vi "Run TDR.vi"(9 "Apply TDR?":bool, 11 "DPE Project File Path":string) -> (0 "error out":errorcluster, 3 "DPI Instrument Name":refnum<k15>)   [LabVIEW 2025, in "Digital Pattern Sequencer.lvclass"]
uses:
  <vilib>/ErrorRing/Error Ring.xnode
  Digital Pattern Sequencer.lvclass
  Digital Pattern Sequencer.lvclass/Digital Pattern Sequencer.ctl
  <vilib>/Utility/error.llb/Error Cluster From Error Code.vi
  <instrlib>/niDigital/niDigital.llb/niDigital Load Specifications Levels and Timing (Single).vi
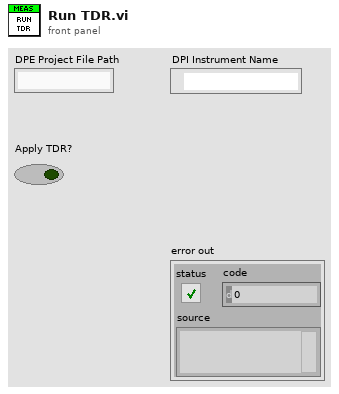
[diagram p1: front panel]
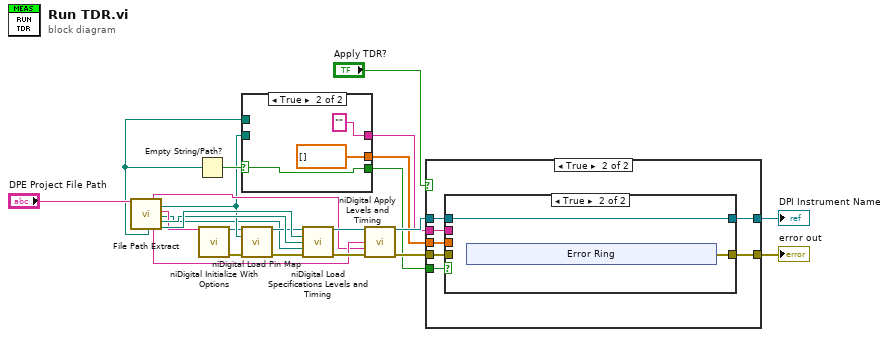
[diagram p0: block diagram]
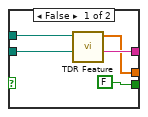
[diagram p2: hidden frame]
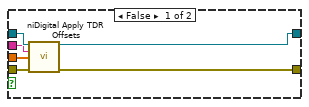
[diagram p4: hidden frame]
diagram:
  n1 = call "File Path Extract.vi"("DPE Project File Path"="DPE Project File Path") -> (".digitdr file path"=w11:path, "Timing path name"=w18:string, "Level path name"=w19:string, ".pinmap file path"=w12:path, "DPI Instrument Name"=w17:string, ".digitiming file path"=w1:path, ".digilevels file path"=w20:path, ".spec file path"=w21:path)  [unwired: 10 in, 1 out]
  n2 = Empty String/Path?(string/path=w11) -> (empty?=w13:bool)
  n3 = call <instrlib>:"niDigital Initialize With Options.vi"("resource name"=w17) -> ("instrument handle"=w6:refnum<k15>, "error out"=w7:errorcluster)  [unwired: 13 in]
  n4 = case shown="True" w13 {
    selector: w13 -> [_ w30]
    tunnel: w12 -> [w29 _]
    tunnel: w11 -> [w28 _]
    tunnel: [w27 "" ("spreadsheet string")] -> w10
    tunnel: [w26 dbl[] [] ("Offset Delay")] -> w9
    tunnel: [FALSE w30] -> w8
    frame False {
      n5 = call "TDR Feature.vi"(".pinmap File Path"=w29, "TDR File Path"=w28) -> ("spreadsheet string"=w27:string, "Offset Delay"=w26:dbl[])  [unwired: 8 in]
    }
    frame True {
    }
  }
  n6 = call <instrlib>:"niDigital Load Pin Map.vi"("instrument handle"=w6, "pin map file"=w12, "error in"=w7) -> ("instrument handle out"=w5:refnum<k15>, "error out"=w4:errorcluster)  [unwired: 11 in]
  n7 = call-poly <instrlib>:"niDigital Load Specifications Levels and Timing.vi"("instrument handle"=w5, "specifications file path"=w21, "levels file path"=w20, "timing file path"=w1, "error in"=w4) -> ("instrument handle out"=w24:refnum<k15>, "error out"=w23:errorcluster)  [unwired: 9 in]
  n8 = call <instrlib>:"niDigital Apply Levels and Timing.vi"("instrument handle"=w24, "levels sheet"=w19, "timing sheet"=w18, "error in"=w23) -> ("instrument handle out"=w16:refnum<k15>, "error out"=w15:errorcluster)  [unwired: 10 in]
  n9 = case shown="True" "Apply TDR?" {
    tunnel: w16 -> [w34 w41]
    tunnel: w15 -> [w33 w40]
    tunnel: [w34 w39] -> w3
    tunnel: [w33 w38] -> w2
    tunnel: w9 -> [_ w37]
    tunnel: w10 -> [_ w36]
    tunnel: w8 -> [_ w35]
    frame False {
    }
    frame True {
      n10 = case shown="True" w35 {
        tunnel: w41 -> [w47 w48]
        tunnel: w40 -> [w46 _]
        tunnel: [w45 w48] -> w39
        tunnel: [w44 w49] -> w38
        tunnel: w37 -> [w43 _]
        tunnel: w36 -> [w42 _]
        frame False {
          n11 = call <instrlib>:"niDigital Apply TDR Offsets.vi"("instrument handle"=w47, "channel list"=w42, "offsets (s)"=w43, "error in"=w46) -> ("instrument handle out"=w45:refnum<k15>, "error out"=w44:errorcluster)  [unwired: 10 in]
        }
        frame True {
          n12 = xnode "Error Ring"() -> ("error out"=w49:errorcluster)
        }
      }
    }
  }
  "DPI Instrument Name" <- w3
  "error out" <- w2
